vi "Reboot Power Reset .vi"() -> (0 "error out":errorcluster, 2 "Result":string, 3 "Result":bool)   [LabVIEW 2021]
uses:
  10054_Control Folder/Support/Relay_no.ctl
panel:
  out "read buffer":string
  out "status":bool
  in  "error in (no error)":errorcluster
  out ".not. x?":bool
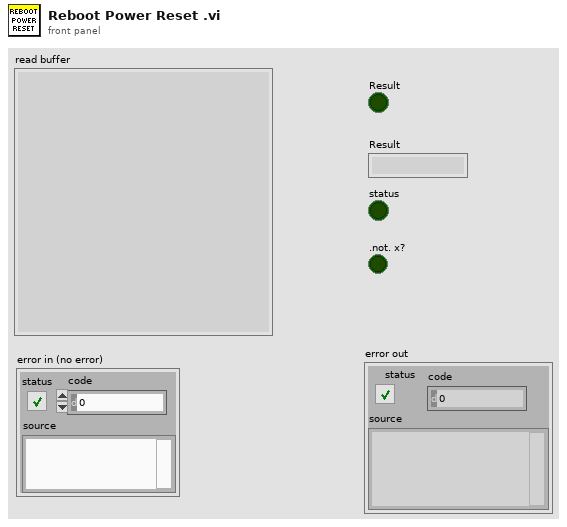
[diagram p1: front panel]
types:
  T1 = typedef "Relay_no.ctl" = enum16{"Init", "write&Read", "PCB Serial Write & Read", "PCB Write SSD & Password", "Read Wifi state", "Reset", "Close"}
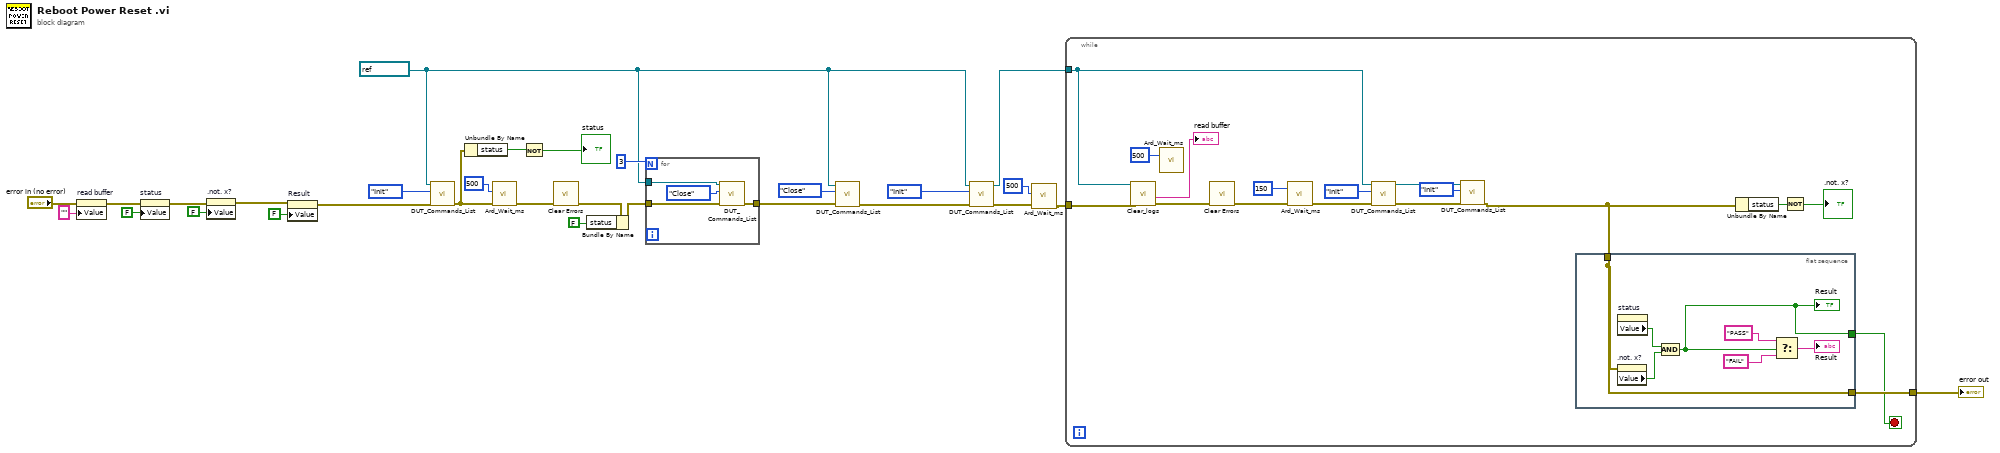
[diagram p0: block diagram]
diagram:
  w12 = refnum<visa-resource-name> "COM3" ("Resource In")
  n1 = property on="read buffer" class="Str"(error in="error in (no error)", "Value"="" ("read buffer")) -> (error out=w3:errorcluster)  [unwired: 1 in, 1 out]
  n2 = property on="status" class="Bool (strict)"(error in=w3, "Value"=FALSE ("status")) -> (error out=w11:errorcluster)  [unwired: 1 in, 1 out]
  n3 = property on=".not. x?" class="Bool (strict)"(error in=w11, "Value"=FALSE (".not. x?")) -> (error out=w10:errorcluster)  [unwired: 1 in, 1 out]
  n4 = property on="Result" class="Bool (strict)"(error in=w10, "Value"=FALSE ("Result")) -> (error out=w9:errorcluster)  [unwired: 1 in, 1 out]
  n5 = call "DUT_Commands_List.vi"("error in"=w9, "Operation"=Relay_no."Init", "Resource In"=w12) -> ("error out"=w26:errorcluster)  [unwired: 6 in, 2 out]
  n6 = Unbundle By Name(w26) -> ("status"=w5:bool)
  n7 = call "Ard_Wait_ms.vi"("error in"=w26, "millisec"=u32 500) -> ("error in 2"=w25:errorcluster)  [unwired: 9 in]
  n8 = Not(x=w5) -> (.not. x?=→"status":bool)
  n9 = call <vilib>:"Clear Errors.vi"("error in (no error)"=w25) -> ("error out"=w23:errorcluster)  [unwired: 5 in, 1 out]
  n10 = Bundle By Name(cluster=w23, "status"=FALSE) -> (w21:errorcluster)
  n11 = for {
    N: 3 -> [_]
    tunnel: w12 -> [w30]
    tunnel: w21 -> [w32]
    tunnel: [w31] -> w19
    n12 = call "DUT_Commands_List.vi"("error in"=w32, "Operation"=Relay_no."Close", "Resource In"=w30) -> ("error out"=w31:errorcluster)  [unwired: 6 in, 2 out]
  }
  n13 = call "DUT_Commands_List.vi"("error in"=w19, "Operation"=Relay_no."Close", "Resource In"=w12) -> ("error out"=w18:errorcluster)  [unwired: 6 in, 2 out]
  n14 = call "DUT_Commands_List.vi"("error in"=w18, "Operation"=Relay_no."Init", "Resource In"=w12) -> ("error out"=w14:errorcluster, "Resource out"=w6:refnum<visa-resource-name>)  [unwired: 6 in, 1 out]
  n15 = call "Ard_Wait_ms.vi"("error in"=w14, "millisec"=u32 500) -> ("error in 2"=w13:errorcluster)  [unwired: 9 in]
  n16 = while {
    tunnel: [w45] -> w29
    tunnel: w13 -> [w42]
    tunnel: w6 -> [w43]
    stop <- w44 stop-if-true
    n17 = call "Clear_logs.vi"("error in (no error)"=w42, "VISA resource name"=w43) -> ("error out"=w36:errorcluster, "read buffer"=→"read buffer":string)  [unwired: 4 in, 2 out]
    n18 = call "Ard_Wait_ms.vi"("millisec"=u32 500) -> ()  [unwired: 10 in, 1 out]
    n19 = call <vilib>:"Clear Errors.vi"("error in (no error)"=w36) -> ("error out"=w35:errorcluster)  [unwired: 5 in, 1 out]
    n20 = call "Ard_Wait_ms.vi"("error in"=w35, "millisec"=u32 150) -> ("error in 2"=w49:errorcluster)  [unwired: 9 in]
    n21 = call "DUT_Commands_List.vi"("error in"=w49, "Operation"=Relay_no."Init", "Resource In"=w43) -> ("error out"=w39:errorcluster, "Resource out"=w38:refnum<visa-resource-name>)  [unwired: 6 in, 1 out]
    n22 = call "DUT_Commands_List.vi"("error in"=w39, "Operation"=Relay_no."Init", "Resource In"=w38) -> ("error out"=w40:errorcluster)  [unwired: 6 in, 2 out]
    n23 = flat-sequence {
      tunnel: w40 -> [w53]
      tunnel: [w53] -> w45
      tunnel: [w52] -> w44
      frame #0 {
        n24 = property on=".not. x?" class="Bool (strict)"(error in=w53) -> ("Value"=w57:bool)  [unwired: 1 in, 2 out]
        n25 = property on="status" class="Bool (strict)"() -> ("Value"=w51:bool)  [unwired: 2 in, 2 out]
        n26 = And(x=w51, y=w57) -> (x .and. y?=w52:bool)
        "Result" <- w52
        n27 = Select(t="PASS", s=w52, f="FAIL") -> (s? t:f=→"Result":string)
      }
    }
    n28 = Unbundle By Name(w40) -> ("status"=w47:bool)
    n29 = Not(x=w47) -> (.not. x?=→".not. x?":bool)
  }
  "error out" <- w29
